vi "Native_GetWhileInfo.vi"() -> ()   [LabVIEW 2024]
panel:
  out "error out":errorcluster caption="错误输出"
  out "terminal_ids":u32[](array[numeric])
  in  "terminal_ids type":u32
  out "diagram_id":u32
  in  "diagram_id type":u32
  in  "loop_id":u32
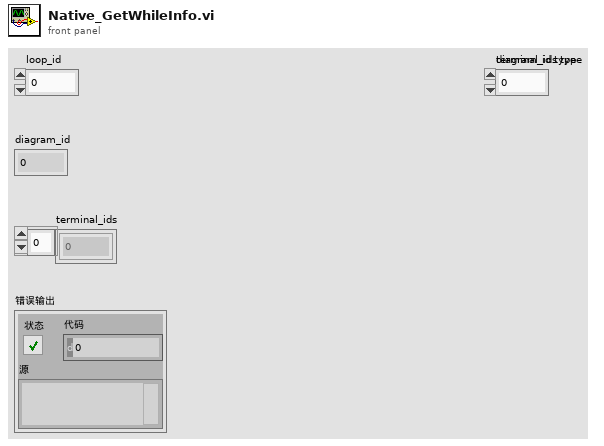
[diagram p1: front panel]
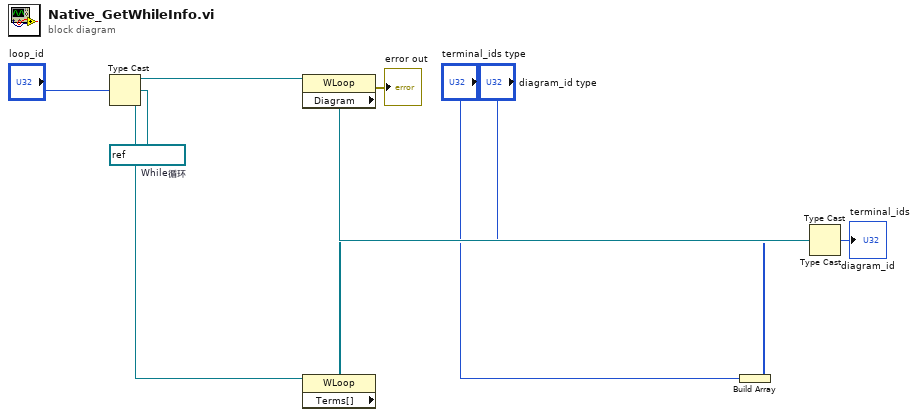
[diagram p0: block diagram]
diagram:
  w10 = refnum<vi> refnum  # While循环
  n1 = Type Cast ("强制类型转换")(type=w10, x="loop_id") -> (*(type *) &x=w9:refnum<vi>)
  n2 = property on="属性节点" class="WLoop"(reference=w9) -> (error out=→"error out":errorcluster, "Diagram"=w8:refnum<vi>)  [unwired: 1 in, 1 out]
  n3 = property on="属性节点" class="WLoop"(reference=w9) -> ("Terms[]"=w5:refnum<vi>[])  [unwired: 1 in, 2 out]
  n4 = Build Array ("创建数组")("terminal_ids type") -> (w3:u32[])
  n5 = Type Cast ("强制类型转换")(type=w3, x=w5) -> (*(type *) &x=→"terminal_ids":u32[])
  n6 = Type Cast ("强制类型转换")(type="diagram_id type", x=w8) -> (*(type *) &x=→"diagram_id":u32)
